vi "Exp - Error handler.vi"(6 "error code in":i32, 7 "InstanceRef":T1, 8 "error in":bool, 9 "cmd (1:set)":i32(ring)=1 items=["init", "set", "get"], 10 "add FuncName (T)":bool=TRUE, 11 "error message in":string) -> (0 "error out":bool, 3 "error message out":string, 4 "error code out":i32)   [LabVIEW 2021]
doc: "Use this VI to declare custom CalcExpress errors in FuncVIs. Refer to the VI help for more details.\n\n::: CalcExpress Toolkit :::\nCopyright (c) 2000-2026 Konstantin Shifershteyn. All rights reserved."
uses:
  cetypes.llb/CalcExpress Instance RefNum.ctl
  cersrc/celveng32.dll
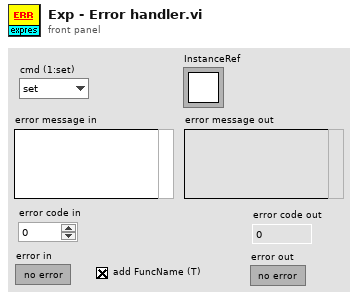
[diagram p1: front panel]
types:
  T1 = typedef "CalcExpress Instance RefNum.ctl" = refnum<k1>
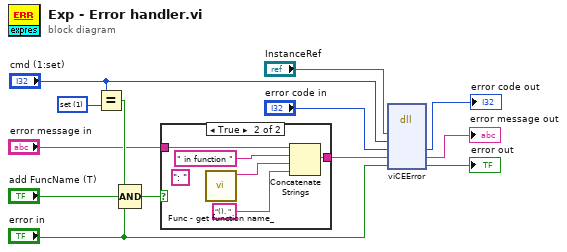
[diagram p0: block diagram]
diagram:
  w4 = 1 items=["init", "set", "get"] ("cmd (def: add)")
  n1 = Equal?(x="cmd (1:set)", y=w4) -> (x = y?=w13:bool)
  n2 = Compound Arithmetic op=AND(w13, "add FuncName (T)", "error in") -> (w12:bool)
  n3 = case shown="True" w12 {
    tunnel: [w14 w16] -> w8
    tunnel: "error message in" -> [w14 w17]
    frame False {
    }
    frame True {
      (unwired) ": "
      n4 = call "Func - get function name_.vi"() -> ("Func name"=w18:string)  [unwired: 9 in, 2 out]
      n5 = Concatenate Strings(w17, " in function ", w18, "(). ") -> (w16:string)
    }
  }
  n6 = dll-call lib="C:/LV Projects/CalcExpress 40 LV2021/vi.lib/addons/CalcExpress/cersrc/celveng*.dll" fn="viCEError"("iRef"="InstanceRef", "cmd"="cmd (1:set)", "errCode"="error code in", "erMsg"=w8, "erf"="error in") -> ("errCode"=→"error code out":i32, "erMsg"=→"error message out":string, "erf"=→"error out":bool)  [unwired: 6 in, 2 out]
